vi "Withdraw Funds.vi"(8 "error in":errorcluster, 9 "Amount":dbl, 10 "Account Number":string, 11 "Accounts File Path":path) -> (0 "error out":errorcluster, 2 "Account":T1, 3 "Sufficient Funds?":bool)   [LabVIEW 2026]
doc: "Withdraws Amount from an account (also used for Fast Cash with Amount 50). The CURRENT balance is read from the accounts file (Get Account.vi). When the balance is at least Amount, Amount is subtracted, the new balance is written with Update Account Balance.vi and Sufficient Funds? is TRUE. Otherwise nothing is written and Sufficient Funds? is FALSE - that is not an error. An account number that is not in the file returns error 5003 and nothing is written. When error in carries an error the file is neither read nor written."
uses:
  Controls/ATM Account.ctl
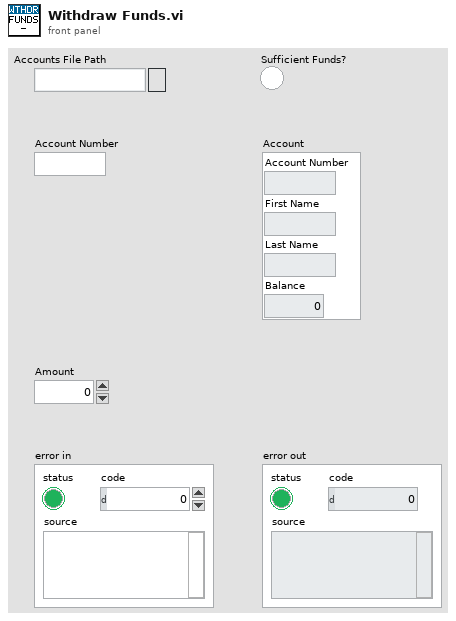
[diagram p1: front panel]
types:
  T1 = typedef "ATM Account.ctl" = cluster{"Account Number":string, "First Name":string, "Last Name":string, "Balance":dbl}
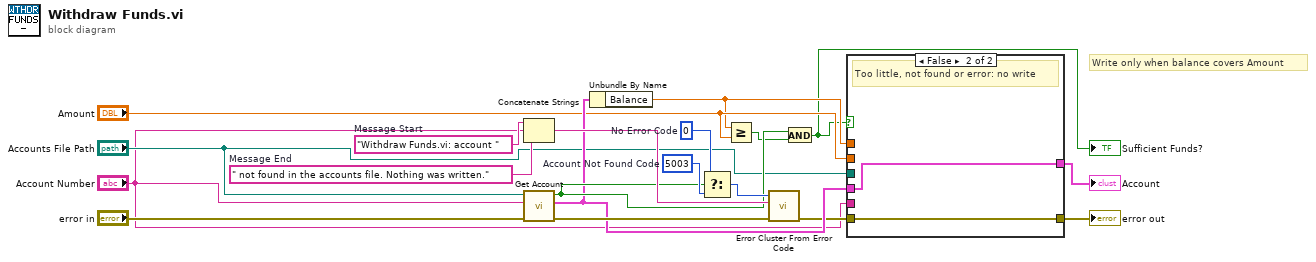
[diagram p0: block diagram]
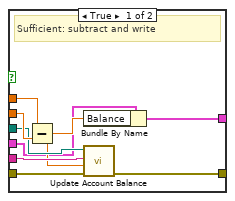
[diagram p2: hidden frame]
diagram:
  w15 = " not found in the accounts file. Nothing was written."  # Message End
  w16 = "Withdraw Funds.vi: account "  # Message Start
  w17 = 5003  # Account Not Found Code
  w18 = 0  # No Error Code
  # "Write only when balance covers Amount"
  n1 = Concatenate Strings(w16, "Account Number", w15) -> (w13:string)
  n2 = call "Get Account.vi"("error in"="error in", "Account Number"="Account Number", "Accounts File Path"="Accounts File Path") -> ("error out"=w12:errorcluster, "Account"=w9:T1, "Account Found?"=w11:bool)  [unwired: 6 in]
  n3 = Unbundle By Name(w9) -> ("Balance"=w4:dbl)
  n4 = Select(t=w18, s=w11, f=w17) -> (s? t:f=w14:i32)
  n5 = Greater Or Equal?(x=w4, y="Amount") -> (x >= y?=w10:bool)
  n6 = call <vilib>:"Error Cluster From Error Code.vi"("error in (no error)"=w12, "error message (\"\")"=w13, "error code (0)"=w14) -> ("error out"=w8:errorcluster)  [unwired: 6 in]
  n7 = And(x=w11, y=w10) -> (x .and. y?=w3:bool)
  "Sufficient Funds?" <- w3
  n8 = case shown="False" w3 {
    tunnel: w9 -> [w22 w30]
    tunnel: w8 -> [w24 w29]
    tunnel: "Accounts File Path" -> [w26 _]
    tunnel: "Account Number" -> [w25 _]
    tunnel: "Amount" -> [w27 _]
    tunnel: w4 -> [w28 _]
    tunnel: [w21 w30] -> w2
    tunnel: [w20 w29] -> w1
    frame True {
      # "Sufficient: subtract and write"
      n9 = Subtract(x=w28, y=w27) -> (x-y=w23:dbl)
      n10 = Bundle By Name(cluster=w22, "Balance"=w23) -> (w21:T1)
      n11 = call "Update Account Balance.vi"("error in"=w24, "New Balance"=w23, "Account Number"=w25, "Accounts File Path"=w26) -> ("error out"=w20:errorcluster)  [unwired: 7 in]
    }
    frame False {
      # "Too little, not found or error: no write"
    }
  }
  "Account" <- w2
  "error out" <- w1
